vi "user32 GetGUIThreadInfo.vi"(0 "thread ID":u32, 5 "cbSize":u32=72, 11 "error in":errorcluster) -> (4 "info":u32[](array[numeric]), 6 "return value":i32, 15 "error out":errorcluster)   [LabVIEW 2020, in "RemoteVI.lvlib"]
doc: "Reads the GUI state of the thread thread ID through user32.dll GetGUIThreadInfo (stdcall, called in any thread) - which window of that thread is active, has the focus, has CAPTURED the mouse, owns a menu ... The GUITHREADINFO structure travels as info, 18 U32 that the function overwrites, with info[0] = cbSize. In 64-bit LabVIEW cbSize is 72 and each HWND is two U32 (low word first): flags [1], hwndActive [2,3], hwndFocus [4,5], hwndCapture [6,7], hwndMenuOwner [8,9], hwndMoveSize [10,11], hwndCaret [12,13], rcCaret [14..17]. In 32-bit LabVIEW cbSize is 48 and each HWND one U32: flags [1], hwndActive [2], hwndFocus [3], hwndCapture [4] ... A wrong cbSize makes the call fail. return value is the Win32 BOOL: non-zero on success, 0 on failure. When error in carries an error the DLL is not called. Generated by scripts\\Build Win32 Wrappers.vi - do not edit by hand, rebuild it."
uses:
  RemoteVI.lvlib
  user32.dll
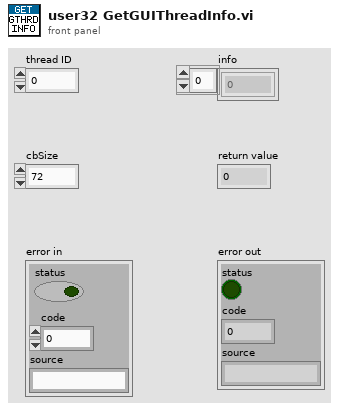
[diagram p1: front panel]
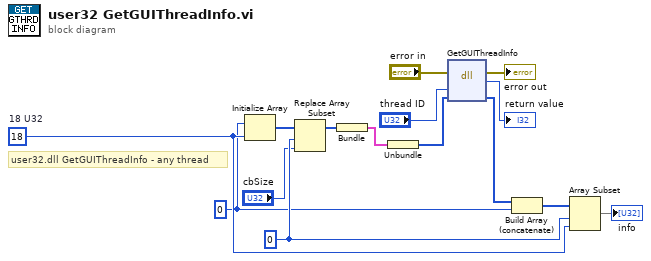
[diagram p0: block diagram]
diagram:
  w11 = 0
  w10 = 18  # 18 U32
  w9 = u32 0
  # "user32.dll GetGUIThreadInfo - any thread"
  n1 = Initialize Array(w9, w10) -> (w12:u32[])
  n2 = Replace Array Subset(array=w12, new element="cbSize", index=w11) -> (w13:u32[])
  n3 = Bundle(w13) -> (w14:cluster{u32[]})  [unwired: 1 in]
  n4 = Unbundle(w14) -> (w2:u32[])
  n5 = dll-call lib="user32.dll" fn="GetGUIThreadInfo"(error in="error in", "idThread"="thread ID", "pgui"=w2) -> (error out=→"error out":errorcluster, →"return value":i32, "pgui"=w1:u32[])  [unwired: 3 in, 1 out]
  n6 = Build Array (concatenate)(w1, w9) -> (w15:u32[])
  n7 = Array Subset(array=w15, index=w11, length=w10) -> (→"info":u32[])
